vi "SendMessageTimeoutW Wrapper Template.vi"(0 "hWnd":u64, 1 "Msg":u32, 2 "wParam":u64, 3 "lParam":i64, 4 "fuFlags":u32=2, 5 "uTimeout":u32=500, 7 "error in":errorcluster) -> (20 "return value":i64, 21 "result":u64, 27 "error out":errorcluster)   [LabVIEW 2020]
doc: "Sends the message Msg to the window hWnd and waits until its thread has processed it, at most uTimeout ms, through user32.dll SendMessageTimeoutW (stdcall, called in any thread). fuFlags 2 = SMTO_ABORTIFHUNG returns at once when the thread is hung. Unlike a posted message a sent one is handled even while LabVIEW's UI thread runs a popup menu's modal loop - RemoteVI Post Input.vi sends WM_CANCELMODE (0x1F) this way to close open LabVIEW popups (measured: posted it is ignored). return value is non-zero on success, 0 on failure or timeout; result is the message's own result. When error in carries an error the DLL is not called. Generated by scripts\\Build Win32 Wrappers.vi - do not edit by hand, rebuild it."
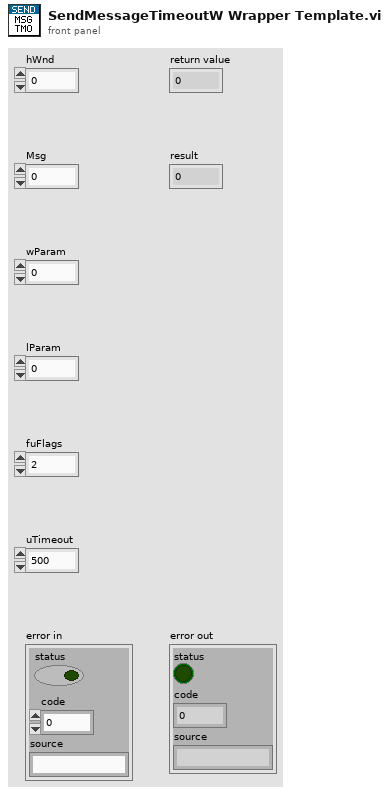
[diagram p1: front panel]
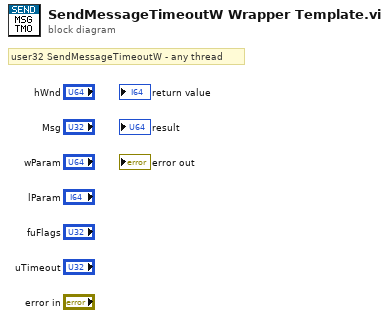
[diagram p0: block diagram]
diagram:
  # "user32 SendMessageTimeoutW - any thread"
